vi "Write FlowGrind.vi"(8 "error in (no error)":errorcluster, 10 "FlowGrind Setting":T1={"Build Profile"=[], "Scale Factor"={"X"=0.002, "Y"=0.025}, "Lap Condition"=100.0, "Supply Pressure"=0.0, "Simulated?"=TRUE} {"Scale Factor"."Y" format="%#_6f"; "Scale Factor"."X" format="%#_4g"; "Build Profile"."Ramp Rate Close" format="%#_f"; "Build Profile"."Null Upper Limit" format="%#_f"; "Build Profile"."Null Lower Limit" format="%#_f"; "Build Profile"."Ramp Rate Far" format="%#_f"; "Build Profile"."Ramp End" format="%#_f"; "Build Profile"."Ramp Start" format="%#_f"}, 11 "XY Plotter configuration in":refnum<class "FlowGrind configuration.lvclass">) -> (0 "error out":errorcluster, 3 "XY Plotter configuration out":refnum<class "FlowGrind configuration.lvclass">)   [LabVIEW 2025, in "Flow Grind.lvlib" / "FlowGrind configuration.lvclass"]
uses:
  FlowGrind configuration.lvclass
  FlowGrind configuration.lvclass/FlowGrind configuration.ctl
  FlowGrind Settings.ctl
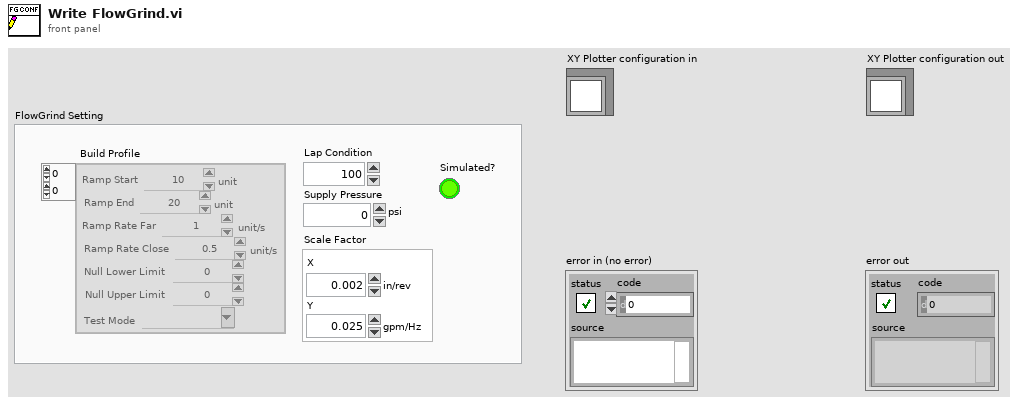
[diagram p1: front panel]
types:
  T1 = typedef "Flow Grind.lvlib/FlowGrind configuration.lvclass/FlowGrind Settings.ctl" = cluster{"Build Profile":cluster{"Ramp Start":dbl, "Ramp End":dbl, "Ramp Rate Far":dbl, "Ramp Rate Close":dbl, "Null Lower Limit":dbl, "Null Upper Limit":dbl, "Test Mode":string}[][], "Scale Factor":cluster{"X":dbl, "Y":dbl}, "Lap Condition":dbl, "Supply Pressure":dbl, "Simulated?":bool}
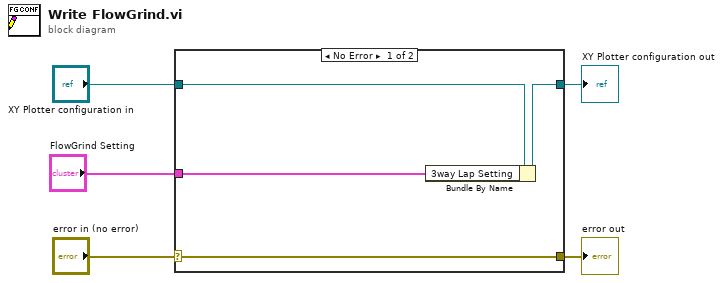
[diagram p0: block diagram]
diagram:
  n1 = case shown="No Error" "error in (no error)" {
    selector: "error in (no error)" -> [w9 w10]
    tunnel: [w9 w10] -> w4
    tunnel: [w7 w11] -> w2
    tunnel: "XY Plotter configuration in" -> [w8 w11]
    tunnel: "FlowGrind Setting" -> [w6 _]
    frame No Error {
      n2 = Bundle By Name(cluster=w8, "3way Lap Setting"=w6) -> (w7:refnum<class "FlowGrind configuration.lvclass">)
    }
    frame Error {
    }
  }
  "error out" <- w4
  "XY Plotter configuration out" <- w2
